vi "Get Alternative List Value.vi"(2 "Current Value":string, 3 "List in":string[](array[string])) -> (0 "Altenative Value":string, 1 "Alternative Available":bool)   [LabVIEW 2020, in "Test.Camera.lvclass"]
uses:
  Test.Camera.lvclass
  <vilib>/Comparison/Equal/Equal Functor/Equal Functor.lvclass
  Test.Camera.lvclass/Test.Camera.ctl
  469305e1-309a-4f6a-b6f2-863a5691b531.vi
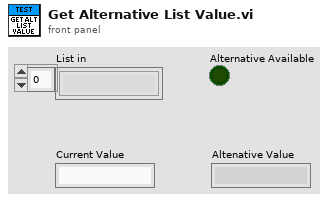
[diagram p1: front panel]
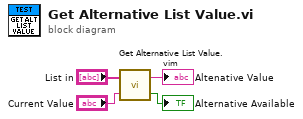
[diagram p0: block diagram]
diagram:
  n1 = call "Get Alternative List Value.vim"("Current Value"="Current Value", "List in"="List in") -> ("Other Value Available"=→"Alternative Available":bool, "Other Value"=→"Altenative Value":string)
